vi "Update Trace Tree.vi"(7 "References":T1, 8 "error in":errorcluster, 10 "Headers":string[](array[string]), 11 "Data IN":string[][](array[string])) -> (0 "error out":errorcluster, 2 "Signals":string[][](table))   [LabVIEW 2025, in "CAN-LIN Raw Bus Capture UI.lvlib"]
doc: "This VI processes the DATA and populates the Frame TREE and the Signal TABLE."
uses:
  CAN-LIN Raw Bus Capture UI.lvlib
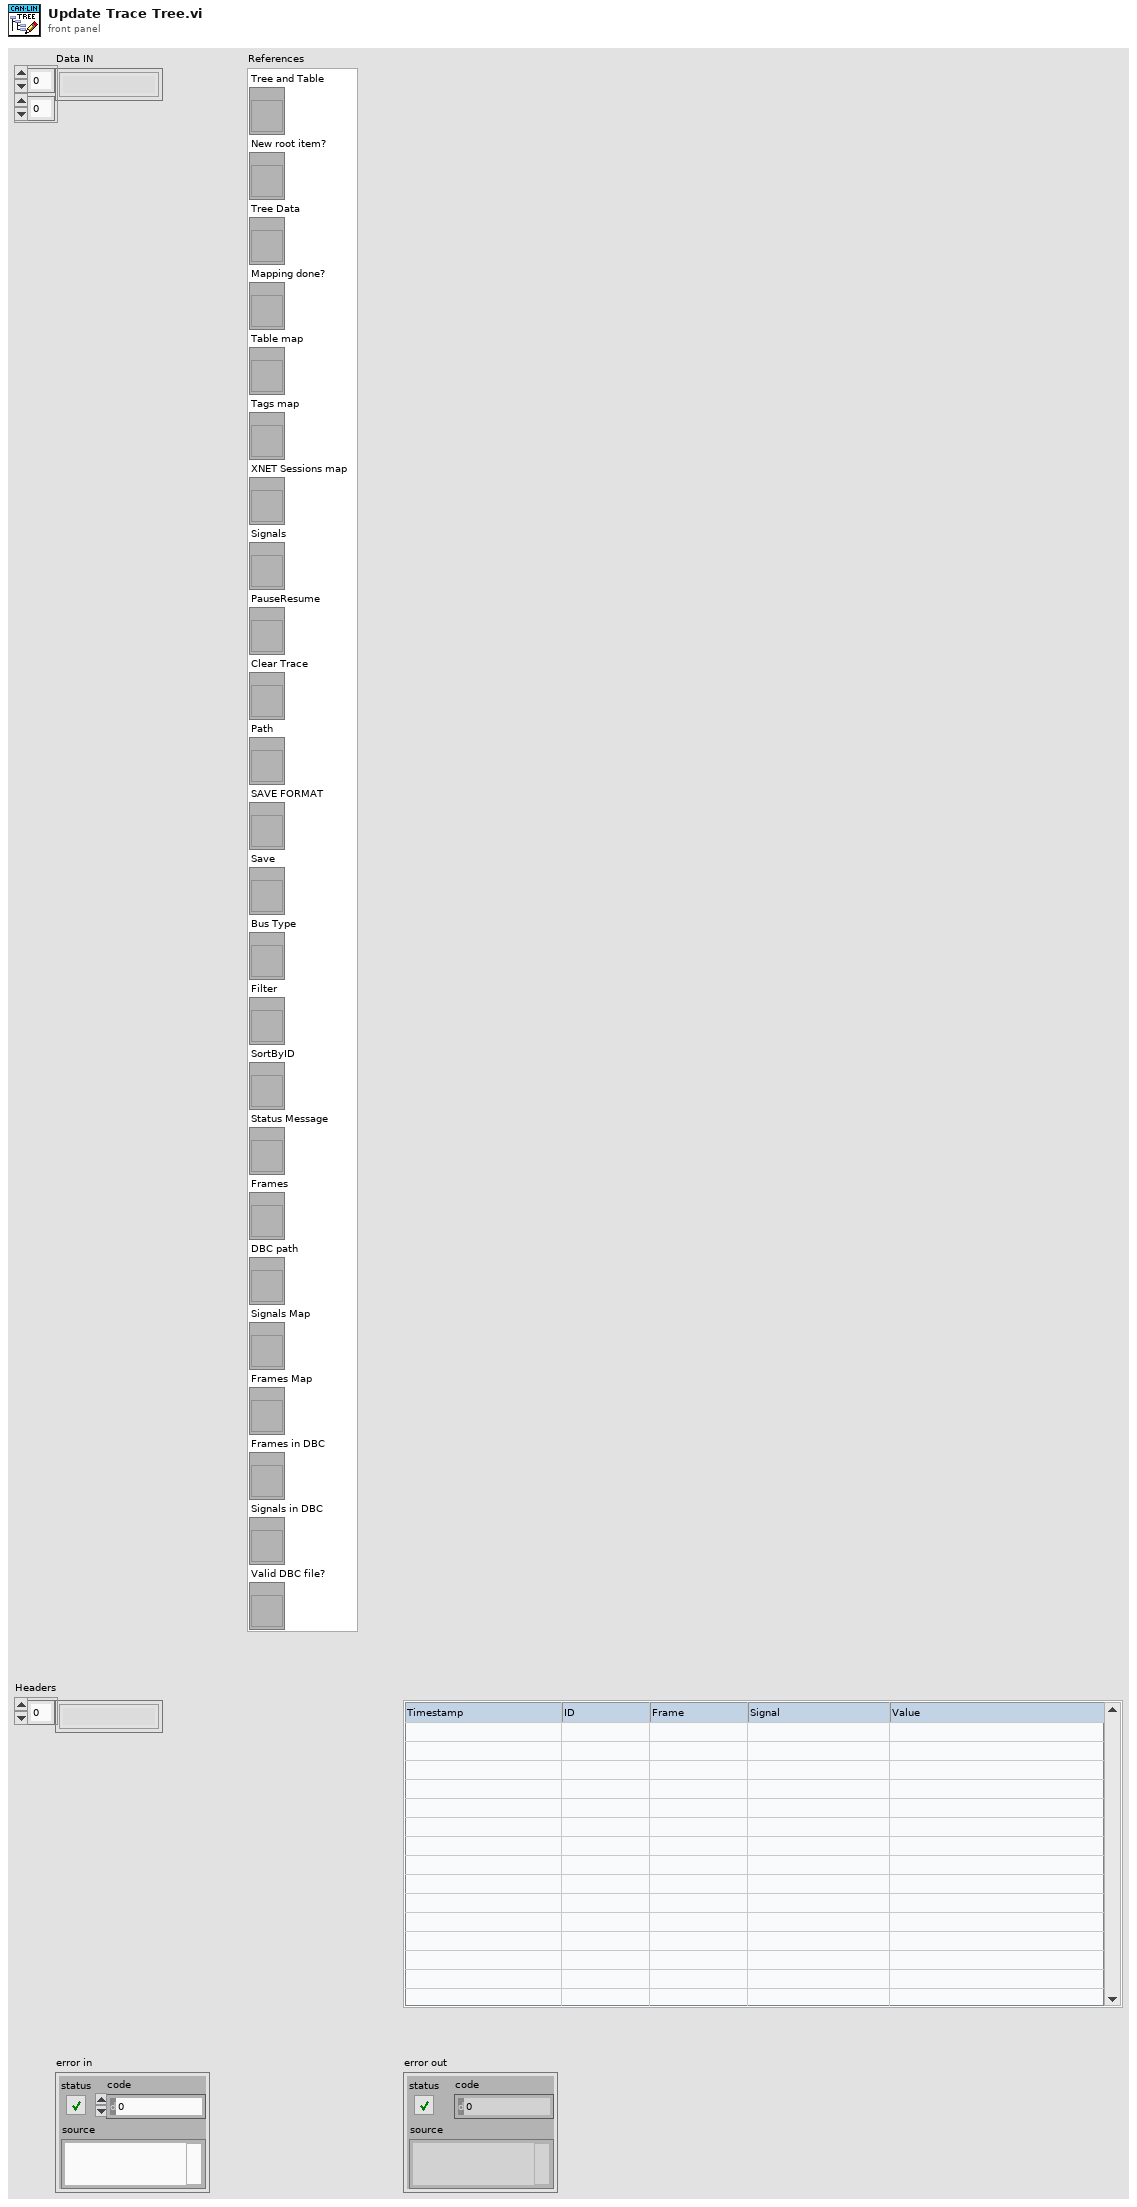
[diagram p1: front panel]
types:
  T1 = cluster{"Tree and Table":refnum<vi>, "New root item?":refnum<vi>, "Tree Data":refnum<vi>, "Mapping done?":refnum<vi>, "Table map":refnum<vi>, "Tags map":refnum<vi>, "XNET Sessions map":refnum<vi>, "Signals":refnum<vi>, "PauseResume":refnum<vi>, "Clear Trace":refnum<vi>, "Path":refnum<vi>, "SAVE FORMAT":refnum<vi>, "Save":refnum<vi>, "Bus Type":refnum<vi>, "Filter":refnum<vi>, "SortByID":refnum<vi>, "Status Message":refnum<vi>, "Frames":refnum<vi>, "DBC path":refnum<vi>, "Signals Map":refnum<vi>, "Frames Map":refnum<vi>, "Frames in DBC":refnum<vi>, "Signals in DBC":refnum<vi>, "Valid DBC file?":refnum<vi>}
  T2 = typedef "XNET Frame CAN.ctl" = cluster{"timestamp":timestamp, "payload":u8[], "identifier":u32, "type":T3, "extended?":bool, "echo?":bool}
  T3 = typedef "XNET Frame Type CAN.ctl" = u8
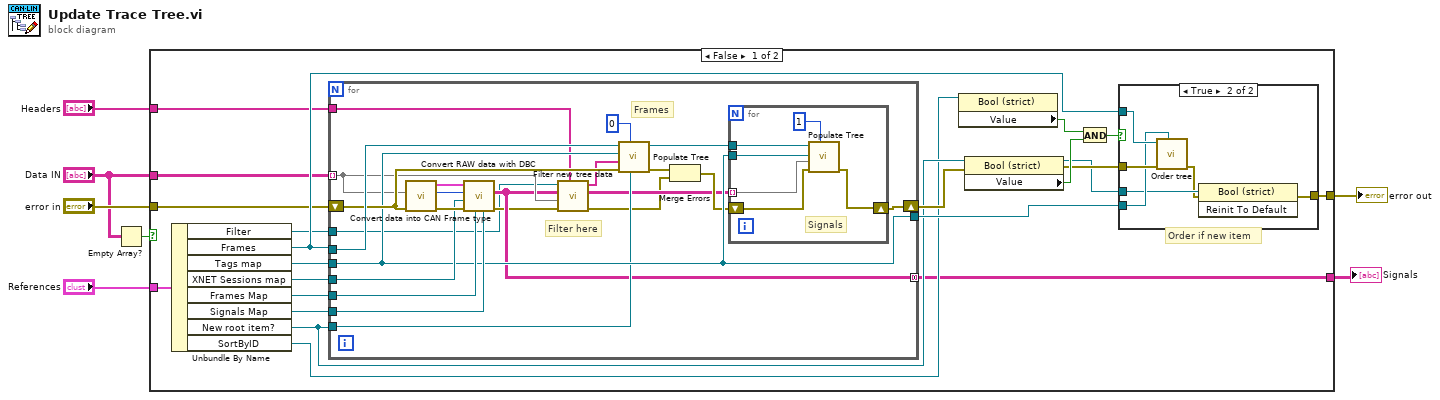
[diagram p0: block diagram]
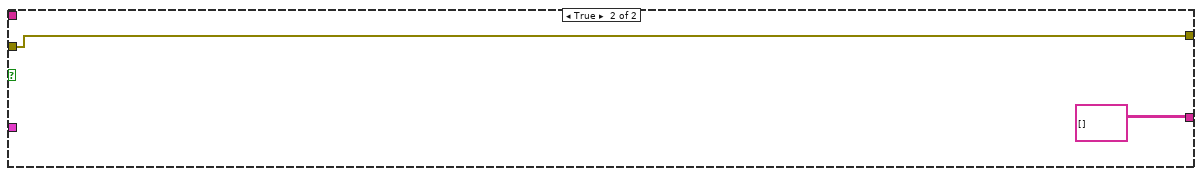
[diagram p3: hidden frame]
diagram:
  n1 = Empty Array?(array="Data IN") -> (empty?=w3:bool)
  n2 = case shown="False" w3 {
    tunnel: [w18 w65] -> w7
    tunnel: "References" -> [w13 _]
    tunnel: "Headers" -> [w12 _]
    tunnel: "Data IN" -> [w11 _]
    tunnel: "error in" -> [w10 w65]
    tunnel: [w8 string[][] [] ("Human Readable DATA")] -> w1
    frame False {
      # "Order if new item"
      n3 = Unbundle By Name(w13) -> ("Filter"=w9:refnum<vi>, "Frames"=w20:refnum<vi>, "Tags map"=w25:refnum<vi>, "XNET Sessions map"=w27:refnum<vi>, "Frames Map"=w26:refnum<vi>, "Signals Map"=w28:refnum<vi>, "New root item?"=w16:refnum<vi>, "SortByID"=w15:refnum<vi>)
      n4 = for {
        tunnel: w11 -> [w36] mode=indexing
        tunnel: w20 -> [w47]
        tunnel: [w33] -> w8 mode=concatenating
        shift-right: [w38] -> w24
        shift-left: w10 -> [w46]
        tunnel: w26 -> [w49]
        tunnel: w28 -> [w48]
        tunnel: w25 -> [w41]
        tunnel: w27 -> [w43]
        tunnel: [w41] -> w19
        tunnel: w16 -> [w40]
        tunnel: w12 -> [w32]
        tunnel: w9 -> [w29]
        # "Filter here"
        # "Frames"
        n5 = call "Convert data into CAN Frame type.vi"("error in"=w46, "Frame"=w36) -> ("error out"=w45:errorcluster, "ID"=w50:u32, "CAN frame"=w44:T2)  [unwired: 7 in]
        n6 = call "Convert RAW data with DBC.vi"("Signals Map"=w48, "Frames Map"=w49, "error in"=w45, "XNET Sessions map"=w43, "ID"=w50, "Frame"=w44) -> ("error out"=w31:errorcluster, "Human Readable DATA"=w33:string[][])  [unwired: 4 in]
        n7 = call "Filter new tree data.vi"("Headers"=w32, "error in"=w31, "Root row"=w36, "Child rows"=w33, "Filter"=w29) -> ("error out"=w30:errorcluster, "Filtered child rows"=w34:string[][], "Filtered root row"=w35:string[])  [unwired: 4 in]
        n8 = call "Populate Tree.vi"("New root item?"=w40, "Indent level"=0 ("Numeric"), "error in"=w46, "Data in"=w35, "Tags map"=w41, "TreeControl in"=w47) -> ("error out"=w39:errorcluster)  [unwired: 5 in]
        n9 = Merge Errors(w39, w30) -> (w37:errorcluster)
        n10 = for {
          tunnel: w34 -> [w51] mode=indexing
          tunnel: w47 -> [w56]
          shift-right: [w54] -> w38
          shift-left: w37 -> [w55]
          tunnel: w41 -> [w53]
          # "Signals"
          n11 = call "Populate Tree.vi"("Indent level"=1, "error in"=w55, "Data in"=w51, "Tags map"=w53, "TreeControl in"=w56) -> ("error out"=w54:errorcluster)  [unwired: 6 in]
        }
      }
      n12 = property class="Bool (strict)"(reference=w15) -> ("Value"=w17:bool)  [unwired: 1 in, 2 out]
      n13 = property class="Bool (strict)"(reference=w16, error in=w24) -> (reference out=w14:refnum<vi>, error out=w21:errorcluster, "Value"=w23:bool)
      n14 = And(x=w17, y=w23) -> (x .and. y?=w22:bool)
      n15 = case shown="True" w22 {
        tunnel: w21 -> [w57 w63]
        tunnel: w20 -> [_ w62]
        tunnel: w19 -> [_ w61]
        tunnel: [w57 w58] -> w18
        tunnel: w14 -> [_ w60]
        frame False {
        }
        frame True {
          n16 = call "Order tree.vi"("Tags map"=w61, "error in"=w63, "TreeControl in"=w62) -> ("error out"=w59:errorcluster)  [unwired: 8 in]
          n17 = invoke class="Bool (strict)" method="Reinit To Default"(reference=w60, error in=w59) -> (error out=w58:errorcluster)  [unwired: 1 in, 2 out]
        }
      }
    }
    frame True {
    }
  }
  "error out" <- w7
  "Signals" <- w1
